vi "DumpFileOpenFile.vi"(9 "Overwrite":bool, 10 "Path":path, 11 "DumpFileState":T1) -> (3 "DumpFileState out":T1)   [LabVIEW 2025]
uses:
  DumpFileState.ctl
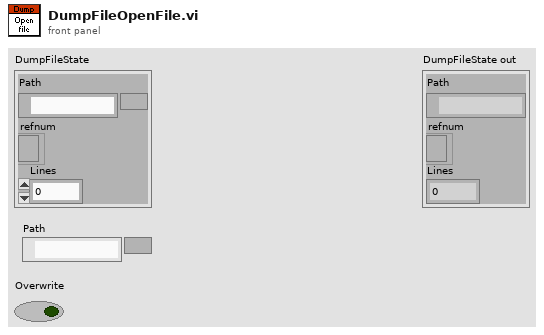
[diagram p1: front panel]
types:
  T1 = typedef "DumpFileState.ctl" = cluster{"Path":path, "refnum":refnum<file>, "Lines":i32}
  T2 = enum16{"open", "replace", "create", "open or create", "replace or create", "replace or create with confirmation"}
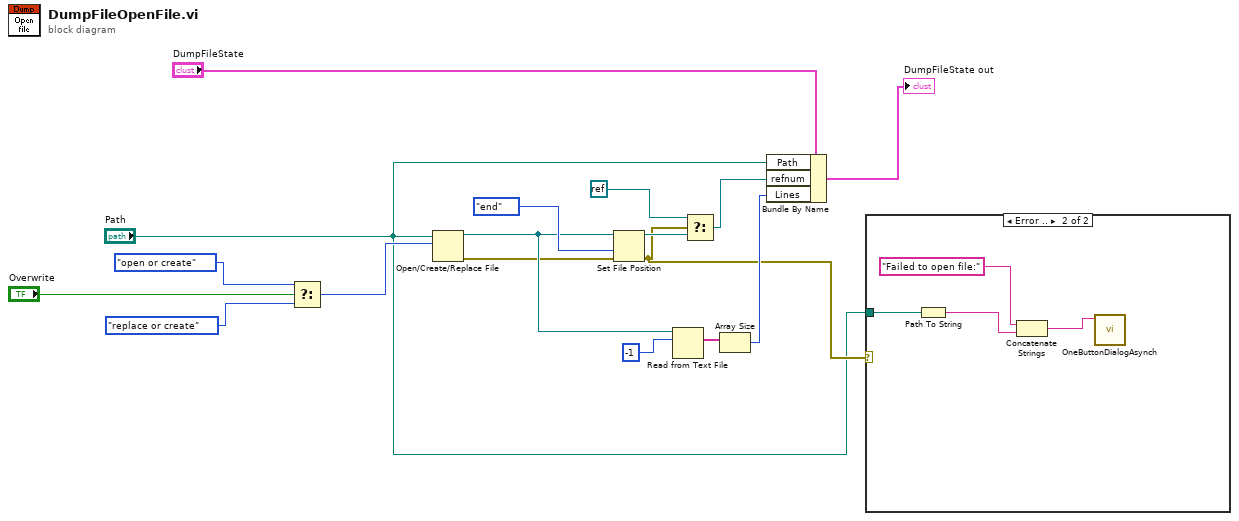
[diagram p0: block diagram]
diagram:
  n1 = Select(t=T2."open or create" ("operation (0:open)"), s="Overwrite", f=T2."replace or create" ("operation (0:open)")) -> (s? t:f=w15:T2)
  n2 = Open/Create/Replace File(file path (use dialog)="Path", operation (0:open)=w15) -> (refnum out=w10:refnum<file>, error out=w6:errorcluster)  [unwired: 4 in, 1 out]
  n3 = Set File Position(refnum=w10, from (0:start)=enum16{"start", "end", "current"}."end", error in=w6) -> (refnum out=w4:refnum<file>, error out=w2:errorcluster)  [unwired: 1 in]
  n4 = Read from Text File(file (use dialog)=w10, count=-1) -> (text=w8:string[])  [unwired: 2 in, 3 out]
  n5 = Select(t=refnum<k0> refnum, s=w2, f=w4) -> (s? t:f=w3:refnum<file>)
  n6 = Array Size(array=w8) -> (size(s)=w7:i32)
  n7 = Bundle By Name(cluster="DumpFileState", "Path"="Path", "refnum"=w3, "Lines"=w7) -> (→"DumpFileState out":T1)
  n8 = case shown="Error .." w2 {
    tunnel: "Path" -> [_ w19]
    frame No Error {
    }
    frame Error {
      n9 = Path To String(path=w19) -> (string=w18:string)
      n10 = Concatenate Strings("Failed to open file:" ("string"), w18) -> (w21:string)
      n11 = call "OneButtonDialogAsynch.vi"("Message to Display"=w21) -> ()  [unwired: 10 in, 1 out]
    }
  }
